vi "Check_Safety.vi"(11 "DI":bool[](array[boolean])) -> (0 "error out":errorcluster, 3 "SafetyOK":bool)   [LabVIEW 2018]
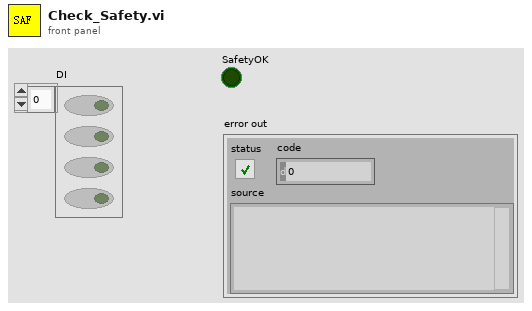
[diagram p1: front panel]
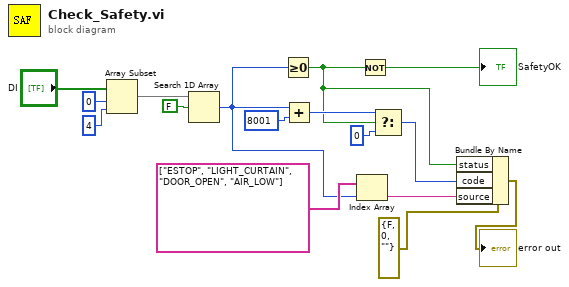
[diagram p0: block diagram]
diagram:
  n1 = Array Subset(array="DI", index=0, length=4) -> (w13:bool[])
  n2 = Search 1D Array(1D array=w13, element=FALSE) -> (index of element=w1:i32)  [unwired: 1 in]
  n3 = Greater Or Equal To 0?(x=w1) -> (x >= 0?=w6:bool)
  n4 = Add(x=w1, y=8001) -> (x+y=w9:i32)
  n5 = Index Array(array=string[] ["ESTOP", "LIGHT_CURTAIN", "DOOR_OPEN", "AIR_LOW"], index=w1) -> (element=w4:string)
  n6 = Not(x=w6) -> (.not. x?=→"SafetyOK":bool)
  n7 = Select(t=w9, s=w6, f=0) -> (s? t:f=w5:i32)
  n8 = Bundle By Name(cluster=errorcluster {"status"=FALSE, "code"=0, "source"=""} ("error out"), "status"=w6, "code"=w5, "source"=w4) -> (→"error out":errorcluster)
